vi "Description.vi"(8 "error in (no error)":errorcluster, 11 "Comparator in":refnum<class "Comparator.lvclass">) -> (0 "error out":errorcluster, 2 "Description":string)   [LabVIEW 2020, in "Comparator.lvclass"]
uses:
  Comparator.lvclass
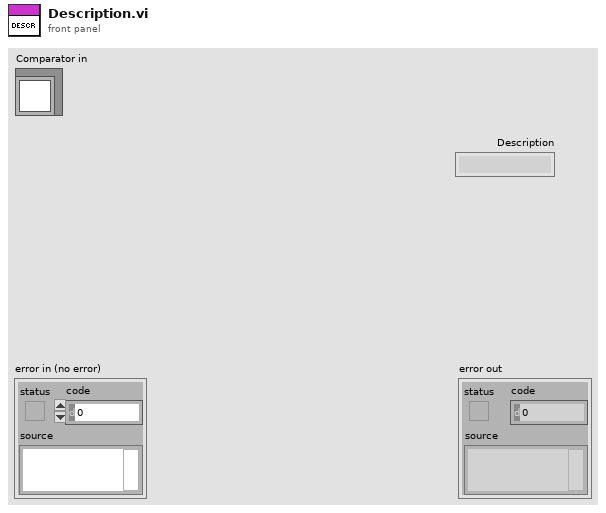
[diagram p1: front panel]
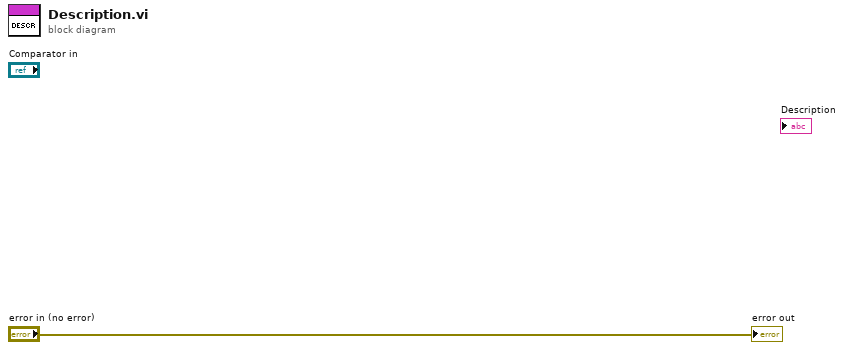
[diagram p0: block diagram]
diagram:
  "error out" <- "error in (no error)"
